vi "myCSVwrite.vi"(5 "响应选项":u8=2, 6 "可用PICO数":u16=2, 7 "注入选项":u8=2, 8 "错误输入（无错误）":errorcluster, 10 "写表结果输入":dbl[][](array[numeric]), 11 "字节流文件输入":refnum<file>) -> (0 "错误输出":errorcluster, 3 "字节流文件输出":refnum<file>)   [LabVIEW 2024]
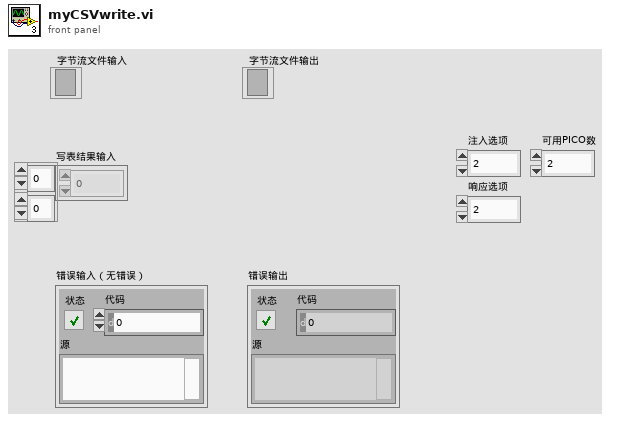
[diagram p1: front panel]
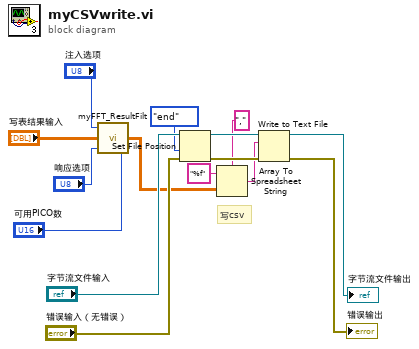
[diagram p0: block diagram]
diagram:
  # "写csv"
  n1 = call "myFFT_ResultFilt.vi"("可用PICO数"="可用PICO数", "响应选项"="响应选项", "写表结果输入"="写表结果输入", "注入选项"="注入选项") -> ("写表结果输出"=w5:dbl[][])  [unwired: 1 in]
  n2 = Set File Position(refnum="字节流文件输入", from (0:start)=enum16{"start", "end", "current"}."end" ("自（0:起始）"), error in="错误输入（无错误）") -> (refnum out=w9:refnum<file>, error out=w10:errorcluster)  [unwired: 1 in]
  n3 = Array To Spreadsheet String(delimiter (Tab)="," ("name (excel)"), array=w5, 3:"%f" ("name (excel)")) -> (spreadsheet string=w8:string)
  n4 = Write to Text File(file (use dialog)=w9, text=w8, error in=w10) -> (refnum out=→"字节流文件输出":refnum<file>, error out=→"错误输出":errorcluster)  [unwired: 1 in, 1 out]
